vi "Load Effect Plugins.vi"() -> (3 "Effect Plugins":refnum<class "Effect Interface.lvclass">[](array[class]))   [LabVIEW 2019, in "Effect Unit.lvclass"]
uses:
  Effect Unit.lvclass
  Plugin Interfaces/Effect Interface/Effect Interface.lvlibp/Effect Interface Class/Effect Interface.lvclass
  <vilib>/Utility/LVLibp/NI_PackedLibraryUtility.lvlib
  Libraries/Audio File Input/Audio File Input.lvlib
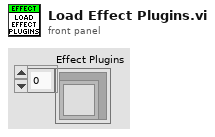
[diagram p1: front panel]
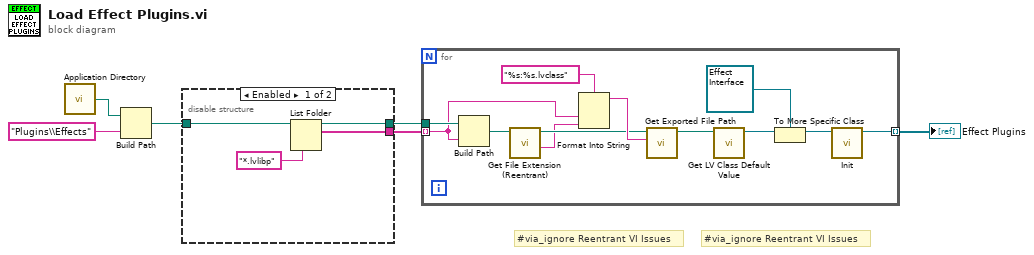
[diagram p0: block diagram]
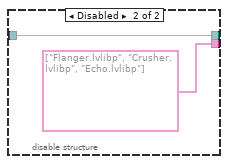
[diagram p2: hidden frame]
diagram:
  # "#via_ignore Reentrant VI Issues"
  # "#via_ignore Reentrant VI Issues"
  n1 = call <vilib>:"Application Directory.vi"() -> ("Application Directory"=w6:path)
  n2 = Build Path(base path=w6, name or relative path="Plugins\\Effects") -> (appended path=w4:path)
  n3 = disable-structure shown="Enabled" {
    disable-tunnel: w4 -> [w10 w11]
    disable-tunnel: [w8 string[] ["Flanger.lvlibp", "Crusher.lvlibp", "Echo.lvlibp"]] -> w3
    disable-tunnel: [w7 w11] -> w2
    frame Enabled {
      n4 = List Folder(path=w10, pattern="*.lvlibp") -> (path out=w7:path, filenames=w8:string[])  [unwired: 2 in, 2 out]
    }
    frame Disabled {
    }
  }
  n5 = for {
    tunnel: w3 -> [w21] mode=indexing
    tunnel: w2 -> [w24]
    tunnel: [w16] -> w1 mode=indexing
    n6 = Build Path(base path=w24, name or relative path=w21) -> (appended path=w15:path)
    n7 = call "Get File Extension (Reentrant).vi"("file"=w15) -> ("filename without extension"=w13:string, "dup file"=w14:path)  [unwired: 6 in, 3 out]
    n8 = Format Into String(format string="%s:%s.lvclass", w21, w13) -> (resulting string=w22:string)  [unwired: 2 in, 1 out]
    n9 = call <vilib>:"Get Exported File Path.vi"("qualified name"=w22, "packed library path"=w14) -> ("path"=w20:path)  [unwired: 8 in, 1 out]
    n10 = call <vilib>:"Get LV Class Default Value.vi"("class path"=w20) -> ("object"=w19:refnum<class>)  [unwired: 9 in, 1 out]
    n11 = To More Specific Class(target class=refnum<class "Effect Interface.lvclass"> refnum ("Effect Interface.lvlibp:Effect Interface.lvclass"), reference=w19) -> (specific class reference=w17:refnum<class "Effect Interface.lvclass">)  [unwired: 1 in, 1 out]
    n12 = call-dynamic "Init.vi"("Effect Interface in"=w17) -> ("Effect Interface out"=w16:refnum<class "Effect Interface.lvclass">)  [unwired: 9 in, 1 out]
  }
  "Effect Plugins" <- w1
